vi "CompVisionUtil_EstimateFieldToRobot.vi"(4 "CameraToRobot":T1={"TRANSLATION3D"={"X"=0.0, "Y"=0.0, "Z"=0.0}, "ROTATION3D"={"Q_quaternion"={"R"=1.0, "V"=[0.0, 0.0, 0.0]}}, "XF"=FALSE} {"TRANSLATION3D"."Z" format="%14.3f"; "TRANSLATION3D"."Y" format="%14.3f"; "TRANSLATION3D"."X" format="%14.3f"}, 5 "cameraHeight_Meters":dbl, 6 "FieldToTarget":T5={"Translation3d"={"X"=0.0, "Y"=0.0, "Z"=0.0}, "Rotation3d"={"Q_quaternion"={"R"=1.0, "V"=[0.0, 0.0, 0.0]}}} {"Translation3d"."Z" format="%14.3f"; "Translation3d"."Y" format="%14.3f"; "Translation3d"."X" format="%14.3f"}, 7 "targetHeight_Meters":dbl, 8 "GyroAngle":T6={"VALUE"=0.0, "COS"=1.0, "SIN"=0.0} {"SIN" format="%13.4f"; "COS" format="%13.4f"; "VALUE" format="%13.4f"}, 9 "TargetYaw":T6={"VALUE"=0.0, "COS"=1.0, "SIN"=0.0} {"SIN" format="%13.4f"; "COS" format="%13.4f"; "VALUE" format="%13.4f"}, 10 "targetPitch_Radians":dbl, 11 "cameraPitch_Radians":dbl) -> (3 "EstimateFieldToRobot":T5={"Translation3d"={"X"=0.0, "Y"=0.0, "Z"=0.0}, "Rotation3d"={"Q_quaternion"={"R"=1.0, "V"=[0.0, 0.0, 0.0]}}} {"Translation3d"."Z" format="%14.3f"; "Translation3d"."Y" format="%14.3f"; "Translation3d"."X" format="%14.3f"})   [LabVIEW 2019, in "Trajectory_Library.lvlib"]
doc: "Estimate the position of the robot in the field.\n\nInputs:\n - CameraHeightMeters -- The physical height of the camera off the floor in meters.\n - TargetHeightMeters -- The physical height of the target off the floor in meters. \n This should be the height of whatever is being targeted (i.e. if the targeting\n region is set to top, this should be the height of the top of the target).\n - CameraPitchRadians -- The pitch of the camera from the horizontal plane in \n radians. Positive values up.\n - TargetPitchRadians -- The pitch of the target in the camera's lens in radians. Positive\n values up.\n - TargetYaw -- Rotation2d representing the observed yaw of the target. Note that this *must* be \n CCW-positive, and Photon returns CW-positive.\n - GyroAngle -- Rotation2d representing he current robot gyro angle, likely from odometry.\n - FieldToTarget -- A Pose3d representing the target position in the field coordinate \n system.\n - CameraToRobot -- The Transform3d position of the robot relative to the camera. If the camera \n was mounted 3 inches behind the \"origin\" (usually physical center) of the\n robot, this would be Transform3d (3 inches, 0 inches, 0 inches, 0 degrees).\n ( Make certain to convert from inches to meters! )\n\nOutputs\n - EstimateFieldToRobot -- The Pose3d position of the robot in the field."
uses:
  Trajectory_Library.lvlib
  TypeDef/ROTATION2D.ctl
  TypeDef/TRANSLATION3D.ctl
  TypeDef/QUATERNION.ctl
  TypeDef/ROTATION3D.ctl
  TypeDef/POSE3D.ctl
  TypeDef/TRANSFORM3D.ctl
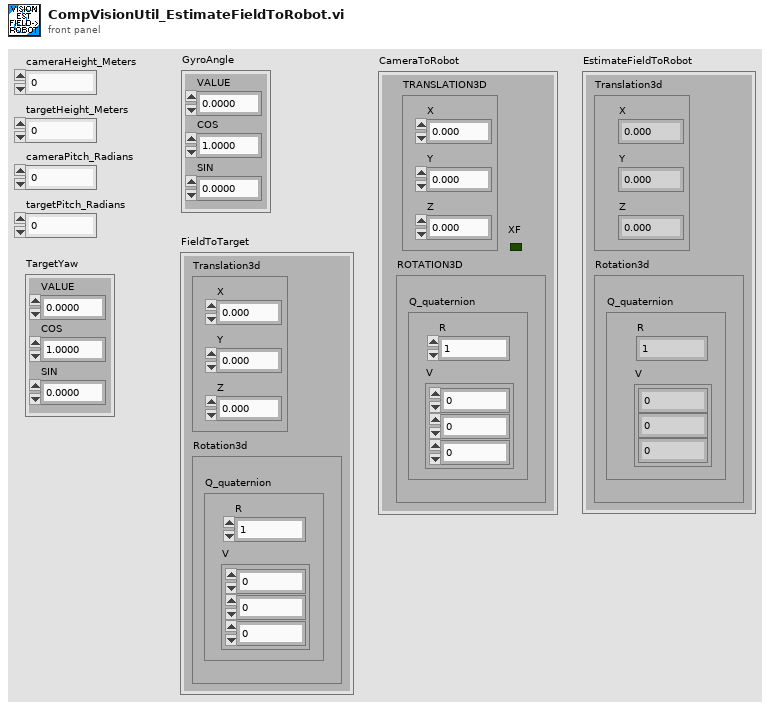
[diagram p1: front panel]
types:
  T1 = typedef "Trajectory_Library.lvlib/TRANSFORM3D.ctl" = cluster{"TRANSLATION3D":T2, "ROTATION3D":T3, "XF":bool}
  T2 = typedef "Trajectory_Library.lvlib/TRANSLATION3D.ctl" = cluster{"X":dbl, "Y":dbl, "Z":dbl}
  T3 = typedef "Trajectory_Library.lvlib/ROTATION3D.ctl" = cluster{"Q_quaternion":T4}
  T4 = typedef "Trajectory_Library.lvlib/QUATERNION.ctl" = cluster{"R":dbl, "V":dbl[]}
  T5 = typedef "Trajectory_Library.lvlib/POSE3D.ctl" = cluster{"Translation3d":T2, "Rotation3d":T3}
  T6 = typedef "Trajectory_Library.lvlib/ROTATION2D.ctl" = cluster{"VALUE":dbl, "COS":dbl, "SIN":dbl}
  T7 = typedef "WPILib_Math.lvlib/POSE3D.ctl" = cluster{"Translation3d":T8, "Rotation3d":T9}
  T8 = typedef "WPILib_Math.lvlib/TRANSLATION3D.ctl" = cluster{"X":dbl, "Y":dbl, "Z":dbl}
  T9 = typedef "WPILib_Math.lvlib/ROTATION3D.ctl" = cluster{"Q_quaternion":T10}
  T10 = typedef "WPILib_Math.lvlib/QUATERNION.ctl" = cluster{"R":dbl, "V":dbl[]}
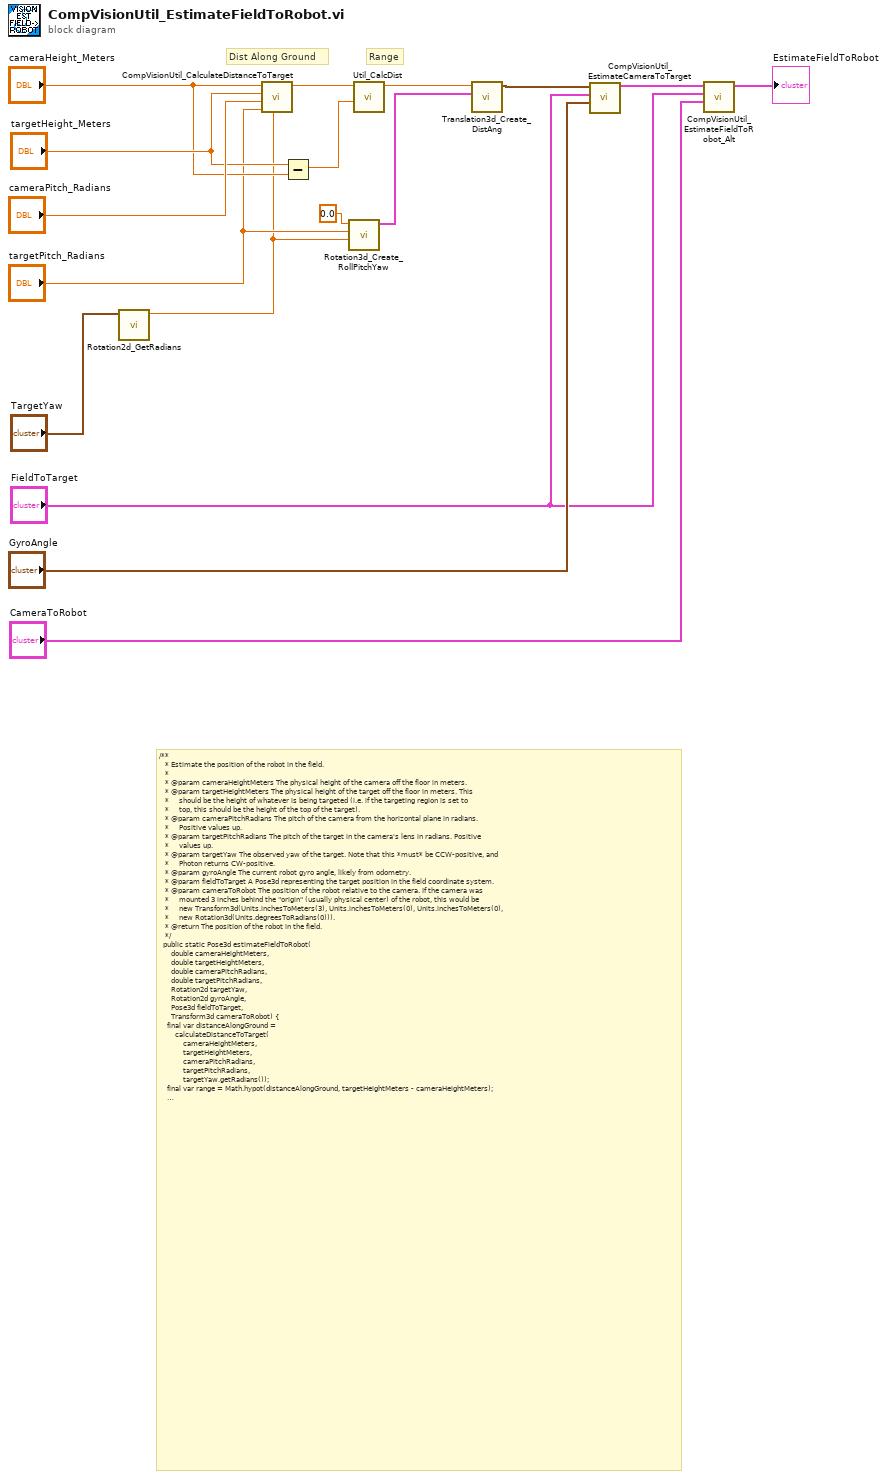
[diagram p0: block diagram]
diagram:
  # "Range"
  # "Dist Along Ground"
  # "/**\n   * Estimate the position of the robot in the field.\n   *\n   * @param cameraHeightMeters The physical height of the camera off the floor in meters.\n   * @param targetHeightMeters The physical height of the target off the floor in meters. This\n   *     should be the height of whatever is being targeted (i.e. if the targeting region is set to\n   *     top, this should be the height of the top of the target).\n   * @param cameraPitchRadians The pitch of the camera from the horizontal plane in radians.\n   *     Positive values up.\n   * @param targetPitchRadians The pitch of the target in the camera's lens in radians. Positive\n   *     values up.\n   * @param targetYaw The observed yaw of the target. Note that this *must* be CCW-positive, and\n   *     Photon returns CW-positive.\n   * @param gyroAngle The current robot gyro angle, likely from odometry.\n   * @param fieldToTarget A Pose3d representing the target position in the field coordinate system.\n   * @param cameraToRobot The position of the robot relative to the camera. If the camera was\n   *     mounted 3 inches behind the \"origin\" (usually physical center) of the robot, this would be\n   *     new Transform3d(Units.inchesToMeters(3), Units.inchesToMeters(0), Units.inchesToMeters(0),\n   *     new Rotation3d(Units.degreesToRadians(0))).\n   * @return The position of the robot in the field.\n   */\n  public static Pose3d estimateFieldToRobot(\n      double cameraHeightMeters,\n      double targetHeightMeters,\n      double cameraPitchRadians,\n      double targetPitchRadians,\n      Rotation2d targetYaw,\n      Rotation2d gyroAngle,\n      Pose3d fieldToTarget,\n      Transform3d cameraToRobot) {\n    final var distanceAlongGround =\n        calculateDistanceToTarget(\n            cameraHeightMeters,\n            targetHeightMeters,\n            cameraPitchRadians,\n            targetPitchRadians,\n            targetYaw.getRadians());\n    final var range = Math.hypot(distanceAlongGround, targetHeightMeters - cameraHeightMeters);\n    return estimateFieldToRobot(\n        estimateCameraToTarget(\n            new Translation3d(\n                range, new Rotation3d(0.0, targetPitchRadians, targetYaw.getRadians())),\n            fieldToTarget,\n            gyroAngle),\n        fieldToTarget,\n        cameraToRobot);\n  }"
  n1 = call "Rotation2d_GetRadians.vi"("in ROTATION"="TargetYaw") -> ("AngleRadians"=w3:dbl)  [unwired: 10 in]
  n2 = call "CompVisionUtil_CalculateDistanceToTarget.vi"("TargetYawRadians"=w3, "targetPitch_Radians"="targetPitch_Radians", "cameraPitch_Radians"="cameraPitch_Radians", "targetHeight_Meters"="targetHeight_Meters", "cameraHeight_Meters"="cameraHeight_Meters") -> ("DistanceToTarget_Meters"=w8:dbl)  [unwired: 6 in]
  n3 = Subtract(x="targetHeight_Meters", y="cameraHeight_Meters") -> (x-y=w7:dbl)
  n4 = call "Rotation3d_Create_RollPitchYaw.vi"("Yaw"=w3, "Pitch"="targetPitch_Radians", "Roll"=0.0) -> ("Rotation3d"=w2:T3)  [unwired: 8 in]
  n5 = call "Util_CalcDist.vi"("Y"=w7, "X"=w8) -> ("DIST"=w6:dbl)  [unwired: 9 in]
  n6 = call "Translation3d_Create_DistAng.vi"("Angle_Rotation3d"=w2, "Distance"=w6) -> ("TRANSLATION3D"=w1:T2)  [unwired: 9 in]
  n7 = call "CompVisionUtil_EstimateCameraToTarget.vi"("GyroAngle"="GyroAngle", "FieldToTarget"="FieldToTarget", "CameraToTargetTranslation"=w1) -> ("EstimateCameraToTarget"=w15:T1)  [unwired: 8 in]
  n8 = call "CompVisionUtil_EstimateFieldToRobot_Alt.vi"("CameraToRobot"="CameraToRobot", "FieldToTarget"="FieldToTarget", "CameraToTarget"=w15) -> ("EstimatedFieldToRobot"=→"EstimateFieldToRobot":T7)  [unwired: 8 in]
